vi "ZM-CP-UDP-openSender.vi"(8 "error in (no error)":errorcluster, 11 "ZM-CP-communication_protocol in":refnum<class "ZM-CP-communication_protocol.lvclass">) -> (0 "error out":errorcluster, 3 "ZM-CP-communication_protocol out":refnum<class "ZM-CP-communication_protocol.lvclass">)   [LabVIEW 2020, in "ZM-CP-UDP-udp_transport.lvlib" / "ZM-CP-UDP-sender.lvclass"]
doc: "Hook of the UDP sender, called by its ZM-CP-init override after Call Parent: opens UDP on any free local port and stores the connection. The class terminals are typed as the parent; Preserve Run-Time Class keeps the sender's class for the override's dynamic output."
uses:
  ZM-CP-UDP-sender.lvclass
  ZM-CP-communication_protocol/ZM-CP-communication_protocol/ZM-CP-communication_protocol.lvclass
  ZM-CP-UDP-sender.lvclass/ZM-CP-UDP-sender.ctl
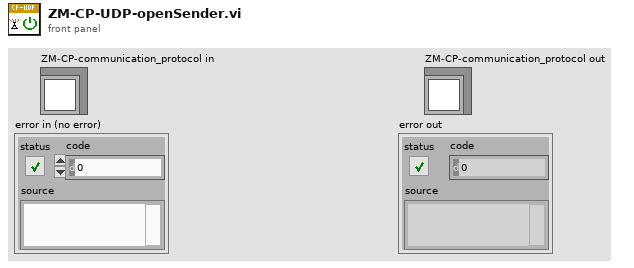
[diagram p1: front panel]
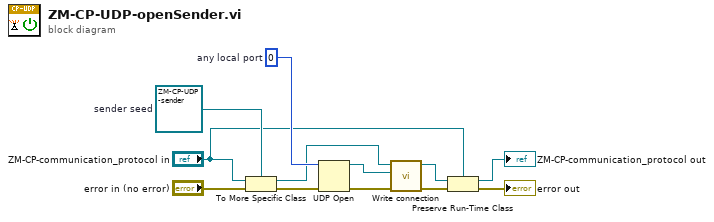
[diagram p0: block diagram]
diagram:
  w10 = u16 0  # any local port
  w11 = refnum<class "ZM-CP-UDP-sender.lvclass"> refnum  # sender seed
  n1 = To More Specific Class(target class=w11, reference="ZM-CP-communication_protocol in", error in="error in (no error)") -> (specific class reference=w7:refnum<class "ZM-CP-UDP-sender.lvclass">, error out=w9:errorcluster)
  n2 = UDP Open(8:w9, 11:w10) -> (port=w6:refnum<k16>, 0:w8:errorcluster)  [unwired: 3 in, 1 out]
  n3 = call "Write connection.vi"("error in (no error)"=w8, "connection"=w6, "ZM-CP-UDP-sender in"=w7) -> ("error out"=w4:errorcluster, "ZM-CP-UDP-sender out"=w5:refnum<class "ZM-CP-UDP-sender.lvclass">)  [unwired: 7 in]
  n4 = Preserve Run-Time Class(object in=w5, error in=w4, 2:"ZM-CP-communication_protocol in") -> (object out=→"ZM-CP-communication_protocol out":refnum<class "ZM-CP-communication_protocol.lvclass">, error out=→"error out":errorcluster)
